vi "test.vi"   [LabVIEW 2021]
uses:
  FirstXNode .xnode
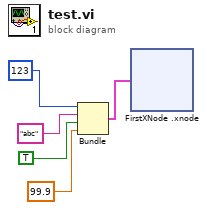
[diagram p0: block diagram]
diagram:
  n1 = Bundle(123, "abc", TRUE, 99.9) -> (w1:cluster{i32, string, bool, dbl})  [unwired: 1 in]
  n2 = xnode "FirstXNode .xnode"("data in"=w1) -> ()  [unwired: 1 out]
